vi "Build Prompt List JSON.vi"(8 "error in":errorcluster, 11 "Prompts":T1(array[cluster])) -> (0 "error out":errorcluster, 3 "prompts json":string)   [LabVIEW 2020, in "MCP Server.lvlib"]
doc: "Builds the prompts array of prompts/list from the registered prompts.\n\nEvery prompt is an object with name, description and arguments. Every argument is an object with name, description and required. required is true for an input that is set to Required on the connector pane of the prompt VI."
uses:
  MCP Server.lvlib
  5517976e-225d-4aae-b967-a015397d673e.vi
  aba5814c-3e0f-4fd3-9e17-57b4859d1148.vi
  a284bf95-fffc-456f-b436-d8ea6015ad6a.vi
  aa18a0ae-7a2f-45a4-bb78-47b2c36abb90.vi
  <vilib>/JDP Science/JSONtext/Variant to JSON Text.vi
  <vilib>/JDP Science/JSONtext/support/Format JSON Array Text.vi
  <vilib>/JDP Science/JSONtext/LVClass Serializer/JSONtext LVClass Serializer.lvclass
  <vilib>/JDP Science/JSONtext/JSONtext.lvlib
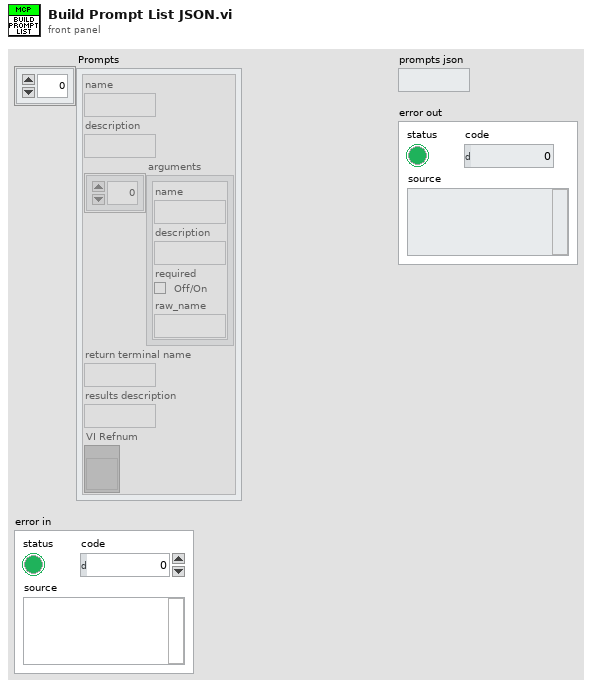
[diagram p1: front panel]
types:
  T1 = cluster{"name":string, "description":string, "arguments":cluster{"name":string, "description":string, "required":bool, "raw_name":string}[], "return terminal name":string, "results description":string, "VI Refnum":refnum<vi>}[]
  T2 = cluster{"name":string, "description":string, "required":bool, "raw_name":string}[]
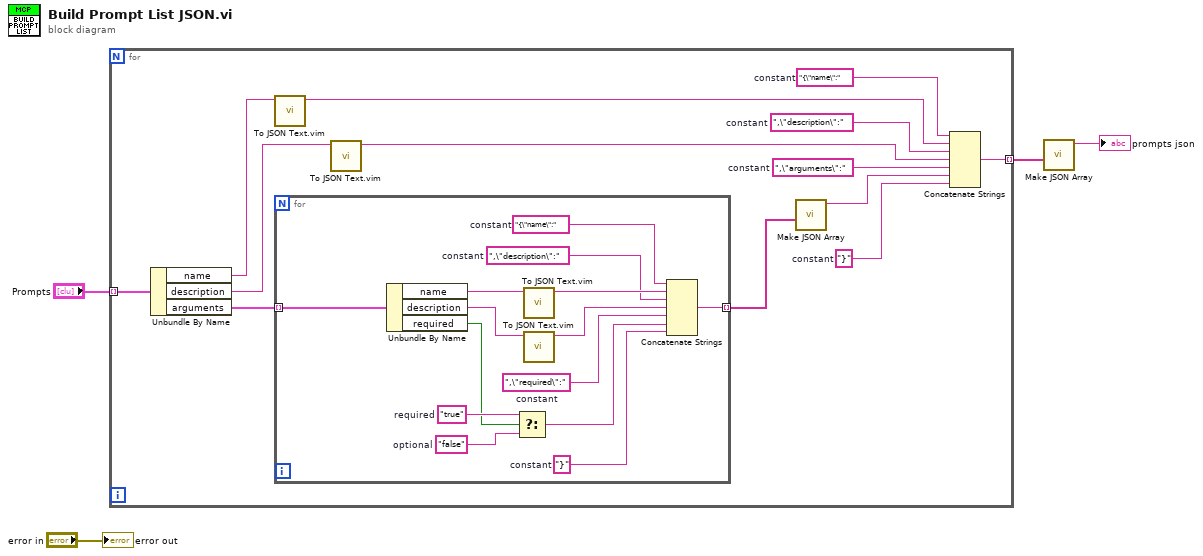
[diagram p0: block diagram]
diagram:
  n1 = for {
    tunnel: "Prompts" -> [w17] mode=indexing
    tunnel: [w5] -> w3 mode=indexing
    w6 = "}"  # constant
    w8 = ",\"arguments\":"  # constant
    w10 = ",\"description\":"  # constant
    w12 = "{\"name\":"  # constant
    n2 = Unbundle By Name(w17) -> ("name"=w14:string, "description"=w13:string, "arguments"=w16:T2)
    n3 = call "To JSON Text.vim"("Anything"=w14) -> ("<JSON>"=w11:string)  [unwired: 9 in, 1 out]
    n4 = for {
      tunnel: w16 -> [w31] mode=indexing
      tunnel: [w18] -> w15 mode=indexing
      w19 = "}"  # constant
      w21 = ",\"required\":"  # constant
      w23 = ",\"description\":"  # constant
      w25 = "{\"name\":"  # constant
      w26 = "false"  # optional
      w28 = "true"  # required
      n5 = Unbundle By Name(w31) -> ("name"=w30:string, "description"=w29:string, "required"=w27:bool)
      n6 = Select(t=w28, s=w27, f=w26) -> (s? t:f=w20:string)
      n7 = call "To JSON Text.vim"("Anything"=w30) -> ("<JSON>"=w24:string)  [unwired: 9 in, 1 out]
      n8 = call "To JSON Text.vim"("Anything"=w29) -> ("<JSON>"=w22:string)  [unwired: 9 in, 1 out]
      n9 = Concatenate Strings(w25, w24, w23, w22, w21, w20, w19) -> (w18:string)
    }
    n10 = call "To JSON Text.vim"("Anything"=w13) -> ("<JSON>"=w9:string)  [unwired: 9 in, 1 out]
    n11 = call <vilib>:"Make JSON Array.vi"("JSON Elements"=w15) -> ("<JSON>"=w7:string)  [unwired: 9 in, 1 out]
    n12 = Concatenate Strings(w12, w11, w10, w9, w8, w7, w6) -> (w5:string)
  }
  n13 = call <vilib>:"Make JSON Array.vi"("JSON Elements"=w3) -> ("<JSON>"=→"prompts json":string)  [unwired: 9 in, 1 out]
  "error out" <- "error in"
